vi "BoolCmd_Recv_Internal.vi"(7 "Command Name":string) -> (0 "error out":errorcluster, 2 "New Request":bool, 3 "Newest Value":bool)   [LabVIEW 2019, in "Trajectory_Library.lvlib"]
uses:
  Trajectory_Library.lvlib
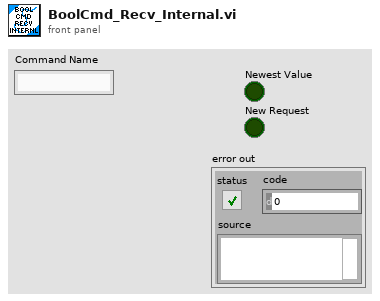
[diagram p1: front panel]
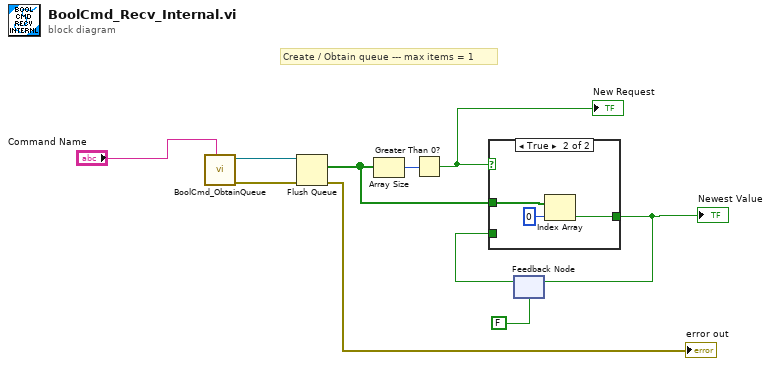
[diagram p0: block diagram]
diagram:
  # "Create / Obtain queue --- max items = 1"
  n1 = call "BoolCmd_ObtainQueue.vi"("Command Name"="Command Name") -> ("error out"=w8:errorcluster, "Queue out"=w9:refnum<queue>)  [unwired: 9 in]
  n2 = Flush Queue(queue=w9, error in (no error)=w8) -> (remaining elements=w5:bool[], error out=→"error out":errorcluster)  [unwired: 1 out]
  n3 = Array Size(array=w5) -> (size(s)=w7:i32)
  n4 = Greater Than 0?(x=w7) -> (x > 0?=w4:bool)
  "New Request" <- w4
  n5 = feedback #1(FALSE) -> (w2:bool)
  n6 = case shown="True" w4 {
    tunnel: w5 -> [_ w14]
    tunnel: [w11 w12] -> w3
    tunnel: w2 -> [w11 _]
    frame False {
    }
    frame True {
      n7 = Index Array(array=w14, index=0) -> (element=w12:bool)
    }
  }
  "Newest Value" <- w3
  n8 = feedback-in #1(w3) -> ()
